vi "Memory Benchmark.vi"(5 "Show Cache Lines (F)":bool, 7 "Show Peak Bandwidth (F)":bool, 9 "Transfers (500)":i32=500, 10 "End Size":u64=50000000 format="%.0pB", 11 "Start Size":u64=1000 format="%.0pB") -> (3 "Memory Bandwidth":cluster{"X":dbl[], "Y":dbl[]}[](graph) caption="Memory Bandwidth Plot")   [LabVIEW 2017]
uses:
  Source/Classes/Pointer/Pointer.lvclass
  Source/Classes/Pointer/Pointer.lvclass/Pointer.ctl
  Source/Classes/Pointer/Copy (No Check).vi
  Source/Classes/Pointer/Check Bounds (Pointer).vi
  Source/Classes/Pointer/Check Null Pointer.vi
  Source/Classes/Pointer/Get Size.vi
  Source/Classes/Pointer/Copy All.vi
  Source/Classes/Pointer/Set Address.vi
  Source/Classes/Pointer/Set Size.vi
  Source/Classes/Pointer/Set Internal.vi
  Source/Classes/Pointer/Clear.vi
  Source/Classes/Pointer/Get Internal.vi
  Source/Classes/Pointer/Errors.vi
  Source/Classes/Pointer/Zone.vi
  Source/Classes/Pointer/Get Address.vi
  Source/Classes/Pointer/Out of Bounds.vi
  Source/Classes/Pointer/Null Pointer.vi
  Source/Classes/Pointer/Is Null.vi
  Source/Classes/Pointer/Clear (No Check).vi
  Source/Classes/Pointer/Check Length.vi
  Source/Classes/Pointer/Create Error.vi
  Source/Classes/Pointer/Write Pointer Size to Error.vi
  Source/Constants/Constants.vi
  Source/Constants/Library Name.vi
  Source/Classes/Pointer/Pointer Error Info.vi
  Source/Constants/Pointer Class Name.vi
  Source/VIs/New Error Cluster.vi
  Source/VIs/New Error Cluster (512B).vi
  Source/VIs/Set Error Status.vi
  Source/VIs/Set Error Code.vi
  Source/VIs/Set Error Source.vi
  Source/VIs/Write String to Source.vi
  Source/VIs/Write Numeric to Source.vi
  Source/VIs/Write Numeric Scalar to Source (Base10 U64).vi
panel:
  out "Peak Throughput":dbl format="%.3pB/s"
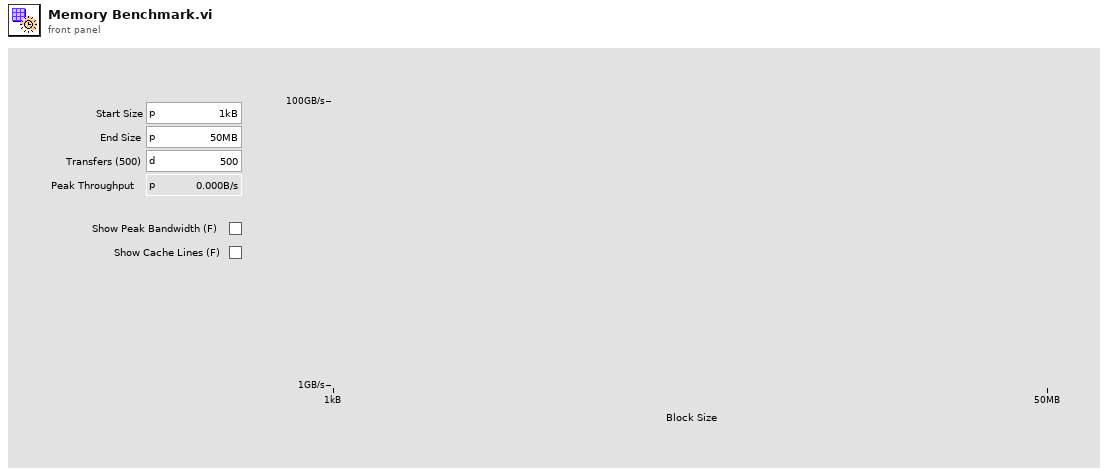
[diagram p1: front panel]
types:
  T1 = typedef "LVAnnotationListTypeDef.ctl" = cluster{"Name":string, "Color":u32, "Style":u8, "Point Style":u8, "Name Visible":bool, "Allow Drag":bool, "Annotation Mode":u32, "Plot":i32, "Index":i32, "Position":cluster{"X":dbl, "Y":dbl}, "X Scale":u32, "Y Scale":u32, "Show Arrow":bool, "Lock Name":bool, "Plot Area":i32, "Label Offset":cluster{"X":dbl, "Y":dbl}}[]
  T2 = cluster{"Name":string, "Color":u32, "Style":u8, "Point Style":u8, "Name Visible":bool, "Allow Drag":bool, "Annotation Mode":u32, "Plot":i32, "Index":i32, "Position":cluster{"X":dbl, "Y":dbl}, "X Scale":u32, "Y Scale":u32, "Show Arrow":bool, "Lock Name":bool, "Plot Area":i32, "Label Offset":cluster{"X":dbl, "Y":dbl}}
  T3 = cluster{"Name":string, "Color":u32, "Style":u8, "Point Style":u8, "Name Visible":bool, "Allow Drag":bool, "Annotation Mode":u32, "Plot":i32, "Index":i32, "Position":cluster{"X":dbl, "Y":dbl}, "X Scale":u32, "Y Scale":u32, "Show Arrow":bool, "Lock Name":bool, "Plot Area":i32, "Label Offset":cluster{"X":dbl, "Y":dbl}}[]
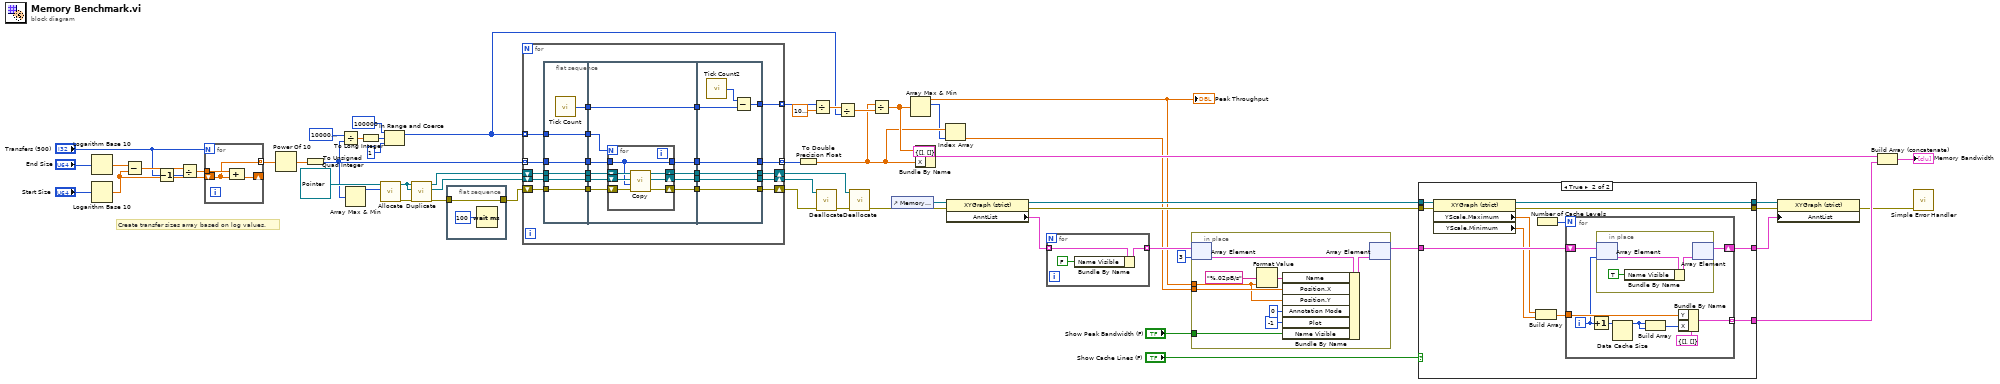
[diagram p0: block diagram]
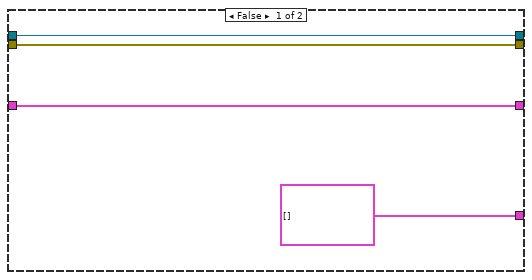
[diagram p2: hidden frame]
diagram:
  # "Create transfer sizes array based on log values."
  n1 = Logarithm Base 10(1:"End Size") -> (0:w55:dbl)
  n2 = Logarithm Base 10(1:"Start Size") -> (0:w52:dbl)
  n3 = Subtract(x=w55, y=w52) -> (x-y=w54:dbl)
  n4 = Decrement(x="Transfers (500)") -> (x-1=w50:i32)
  n5 = Divide(x=w54, y=w50) -> (x/y=w53:dbl)
  n6 = for {
    N: "Transfers (500)" -> [_]
    tunnel: w53 -> [w60]
    shift-right: [w59] -> _
    shift-left: w52 -> [w58]
    tunnel: [w58] -> w49 mode=indexing
    n7 = Compound Arithmetic op=ADD(w60, w58) -> (w59:dbl)
  }
  n8 = Power Of 10(x=w49) -> (10^x=w48:dbl[])
  n9 = To Unsigned Quad Integer(1:w48) -> (0:w1:u64[])
  n10 = Divide(x=u64 100000000, y=w1) -> (x/y=w42:dbl[])
  n11 = Array Max & Min(array=w1) -> (max value=w8:u64)  [unwired: 3 out]
  n12 = To Long Integer(number=w42) -> (32bit integer=w41:i32[])
  n13 = call "Allocate.vi"("size"=w8, "Pointer type"=refnum<class "Pointer.lvclass"> refnum ("Pointer in")) -> ("error out"=w38:errorcluster, "Pointer out"=w3:refnum<class "Pointer.lvclass">)  [unwired: 8 in]
  n14 = In Range and Coerce(upper limit=100000, x=w41, lower limit=1) -> (coerced(x)=w22:i32[])  [unwired: 1 out]
  n15 = call "Duplicate.vi"("error in (no error)"=w38, "new Pointer type"=w3, "Pointer in"=w3) -> ("error out"=w28:errorcluster, "new Pointer"=w5:refnum<class "Pointer.lvclass">, "Pointer out"=w4:refnum<class "Pointer.lvclass">)  [unwired: 6 in]
  n16 = flat-sequence {
    tunnel: w28 -> [w62]
    tunnel: [w62] -> w27
    frame #0 {
      n17 = Wait (ms)(milliseconds to wait=u32 100) -> ()  [unwired: 1 out]
    }
  }
  n18 = for {
    shift-right: [w67] -> w36
    shift-left: w5 -> [w71]
    shift-right: [w66] -> w34
    shift-left: w4 -> [w70]
    shift-right: [w68] -> w37
    shift-left: w27 -> [w69]
    tunnel: [w65] -> w32 mode=indexing
    tunnel: w1 -> [w64] mode=indexing
    tunnel: [w63] -> w29 mode=indexing
    tunnel: w22 -> [w72] mode=indexing
    n19 = flat-sequence {
      tunnel: [w89] -> w83
      tunnel: [w88] -> w82
      tunnel: [w87] -> w81
      tunnel: [w86] -> w80
      tunnel: [w85] -> w79
      tunnel: [w84] -> w78
      tunnel: w70 -> [w89]
      tunnel: w71 -> [w88]
      tunnel: w69 -> [w87]
      tunnel: w64 -> [w86]
      tunnel: w72 -> [w85]
      tunnel: w83 -> [w99]
      tunnel: w82 -> [w90]
      tunnel: w81 -> [w98]
      tunnel: w80 -> [w97]
      tunnel: w79 -> [w93]
      tunnel: w78 -> [w92]
      tunnel: [w92] -> w77
      tunnel: [w96] -> w76
      tunnel: [w95] -> w75
      tunnel: [w94] -> w74
      tunnel: [w91] -> w73
      tunnel: w77 -> [w112]
      tunnel: w76 -> [w111]
      tunnel: w75 -> [w110]
      tunnel: w74 -> [w109]
      tunnel: w73 -> [w108]
      tunnel: [w111] -> w68
      tunnel: [w110] -> w66
      tunnel: [w109] -> w67
      tunnel: [w108] -> w63
      tunnel: [w107] -> w65
      frame #0 {
        n20 = call "Tick Count"() -> ("Tick Count(uSec)"=w84:u32)
      }
      frame #1 {
        n21 = for {
          N: w93 -> [_]
          shift-right: [w103] -> w96
          shift-left: w98 -> [w104]
          shift-right: [w102] -> w95
          shift-left: w99 -> [w106]
          shift-right: [w101] -> w94
          shift-left: w90 -> [w105]
          tunnel: w97 -> [w100]
          tunnel: [w100] -> w91
          n22 = call "Copy.vi"("error in (no error)"=w104, "size"=w100, "dst Pointer in"=w105, "src Pointer in"=w106) -> ("error out"=w103:errorcluster, "dst Pointer out"=w101:refnum<class "Pointer.lvclass">, "src Pointer out"=w102:refnum<class "Pointer.lvclass">)  [unwired: 4 in, 1 out]
        }
      }
      frame #2 {
        n23 = call "Tick Count2"() -> ("Tick Count(uSec)"=w113:u32)
        n24 = Subtract(x=w113, y=w112) -> (x-y=w107:u32)
      }
    }
  }
  n25 = To Double Precision Float(number=w29) -> (double precision float=w26:dbl[])
  n26 = Divide(x=w32, y=1000000.0) -> (x/y=w31:dbl[])
  n27 = call "Deallocate.vi"("error in (no error)"=w37, "Pointer"=w36) -> ("error out"=w35:errorcluster)  [unwired: 8 in, 1 out]
  n28 = Divide(x=w31, y=w22) -> (x/y=w30:dbl[])
  n29 = call "Deallocate.vi"("error in (no error)"=w35, "Pointer"=w34) -> ("error out"=w12:errorcluster)  [unwired: 8 in, 1 out]
  n30 = Divide(x=w26, y=w30) -> (x/y=w47:dbl[])
  n31 = control-ref of="Memory Bandwidth"() -> (w20:refnum<vi>)
  n32 = Array Max & Min(array=w47) -> (max value=w14:dbl, max index (indices)=w24:i32)  [unwired: 2 out]
  "Peak Throughput" <- w14
  n33 = Bundle By Name(cluster=cluster{"X":dbl[], "Y":dbl[]} {"X"=[], "Y"=[]}, "Y"=w47, "X"=w26) -> (w45:cluster{"X":dbl[], "Y":dbl[]})
  n34 = Index Array(array=w26, index=w24) -> (element=w13:dbl)
  n35 = property class="XYGraph (strict)"(reference=w20, error in=w12) -> (reference out=w15:refnum<vi>, error out=w16:errorcluster, "AnntList"=w19:T1)
  n36 = for {
    tunnel: w19 -> [w115] mode=indexing
    tunnel: [w114] -> w17 mode=indexing
    n37 = Bundle By Name(cluster=w115, "Name Visible"=FALSE) -> (w114:T2)
  }
  n38 = in-place {
    in-place-border: w14 -> [w117]
    in-place-border: w13 -> [w121]
    in-place-border: "Show Peak Bandwidth (F)" -> [w118]
    n39 = in-place-array #1(w17, 3) -> (w125:T2)
    n40 = Format Value(format string="%.02pB/s", value (0)=w117) -> (output string=w123:string)  [unwired: 1 in]
    n41 = Bundle By Name(cluster=w125, "Name"=w123, "Position.X"=w121, "Position.Y"=w117, "Annotation Mode"=u32 0, "Plot"=-1, "Name Visible"=w118) -> (w122:T2)
    n42 = in-place-array #1(w122) -> (w21:T3)  [unwired: 1 out]
  }
  n43 = case shown="True" "Show Cache Lines (F)" {
    tunnel: [cluster{"X":dbl[], "Y":dbl[]}[] [] w138] -> w7
    tunnel: w15 -> [w126 w137]
    tunnel: w21 -> [w127 w136]
    tunnel: w16 -> [w128 w135]
    tunnel: [w128 w132] -> w11
    tunnel: [w126 w131] -> w10
    tunnel: [w127 w130] -> w9
    frame False {
    }
    frame True {
      n44 = property class="XYGraph (strict)"(reference=w137, error in=w135) -> (reference out=w131:refnum<vi>, error out=w132:errorcluster, "YScale.Maximum"=w134:dbl, "YScale.Minimum"=w133:dbl)
      n45 = Build Array(w134, w133) -> (w139:dbl[])
      n46 = Number of Cache Levels() -> (w140:i32)
      n47 = for {
        N: w140 -> [_]
        tunnel: w139 -> [w145]
        tunnel: [w144] -> w138 mode=indexing
        shift-right: [w142] -> w130
        shift-left: w136 -> [w143]
        i -> [w141]
        n48 = Increment(x=w141) -> (x+1=w149:i32)
        n49 = in-place {
          n50 = in-place-array #2(w143, w141) -> (w152:T2)
          n51 = Bundle By Name(cluster=w152, "Name Visible"=TRUE) -> (w151:T2)
          n52 = in-place-array #2(w151) -> (w142:T3)  [unwired: 1 out]
        }
        n53 = Data Cache Size(0:w149) -> (4:w147:i32)  [unwired: 1 out]
        n54 = Build Array(w147, w147) -> (w146:i32[])
        n55 = Bundle By Name(cluster=cluster{"X":dbl[], "Y":dbl[]} {"X"=[], "Y"=[]}, "Y"=w145, "X"=w146) -> (w144:cluster{"X":dbl[], "Y":dbl[]})
      }
    }
  }
  n56 = property class="XYGraph (strict)"(reference=w10, error in=w11, "AnntList"=w9) -> (error out=w6:errorcluster)  [unwired: 1 out]
  n57 = Build Array (concatenate)(w45, w7) -> (→"Memory Bandwidth":cluster{"X":dbl[], "Y":dbl[]}[])
  n58 = call <vilib>:"Simple Error Handler.vi"("error in (no error)"=w6) -> ()  [unwired: 4 in, 5 out]
